vi "base info txt ransfer.vi"(11 "Base All Composition_edit":T1(array[cluster])) -> (3 "transposed array":string[][](array[string]))   [LabVIEW 2018]
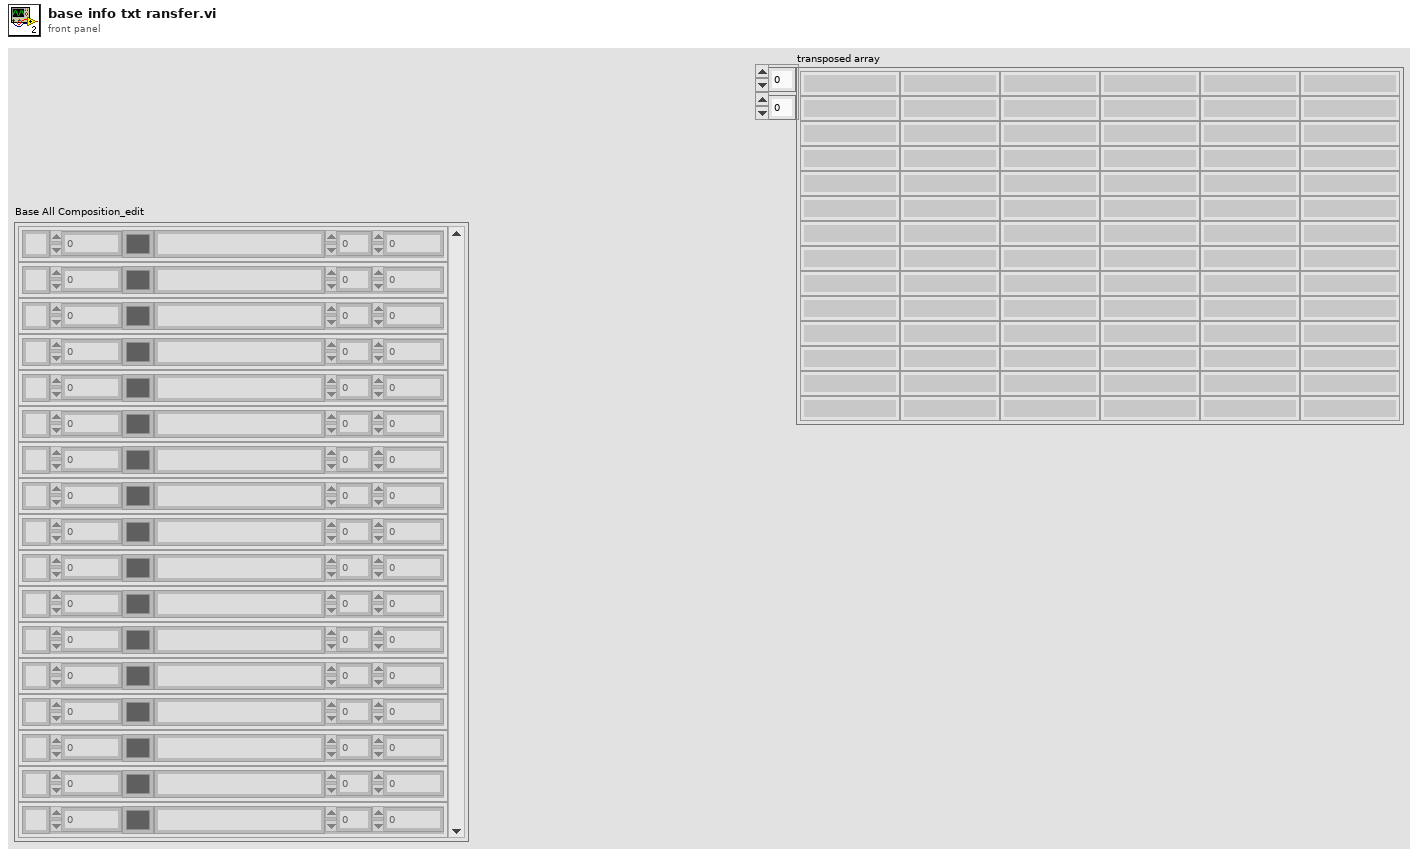
[diagram p1: front panel]
types:
  T1 = cluster{"Name":string, "Value":dbl, "Color":u32, "Name 2":string, "Value 2":dbl, "Value 3":dbl}[]
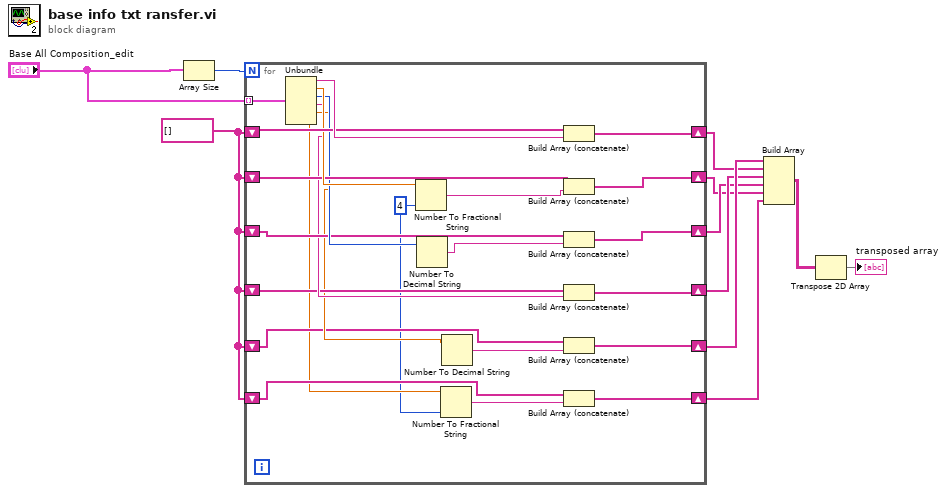
[diagram p0: block diagram]
diagram:
  w9 = string[] []
  n1 = Array Size(array="Base All Composition_edit") -> (size(s)=w11:i32)
  n2 = for {
    N: w11 -> [_]
    tunnel: "Base All Composition_edit" -> [w35] mode=indexing
    shift-right: [w34] -> w6
    shift-left: w9 -> [w32]
    shift-right: [w29] -> w3
    shift-left: w9 -> [w28]
    shift-right: [w25] -> w4
    shift-left: w9 -> [w24]
    shift-right: [w23] -> w5
    shift-left: w9 -> [w21]
    shift-right: [w20] -> w7
    shift-left: w9 -> [w16]
    shift-right: [w19] -> w8
    shift-left: w9 -> [w15]
    w13 = i16 4 ("precision (6)")
    n3 = Unbundle(w35) -> ("Name"=w33:string, "Value"=w31:dbl, "Color"=w27:u32, "Name 2"=w22:string, "Value 2"=w18:dbl, "Value 3"=w14:dbl)
    n4 = Number To Fractional String(number=w31, precision (6)=w13) -> (F-format string=w30:string)  [unwired: 2 in]
    n5 = Number To Decimal String(number=w27) -> (decimal integer string=w26:string)  [unwired: 1 in]
    n6 = Number To Fractional String(number=w14, precision (6)=w13) -> (F-format string=w12:string)  [unwired: 2 in]
    n7 = Number To Decimal String(number=w18) -> (decimal integer string=w17:string)  [unwired: 1 in]
    n8 = Build Array (concatenate)(w32, w33) -> (w34:string[])
    n9 = Build Array (concatenate)(w28, w30) -> (w29:string[])
    n10 = Build Array (concatenate)(w24, w26) -> (w25:string[])
    n11 = Build Array (concatenate)(w21, w22) -> (w23:string[])
    n12 = Build Array (concatenate)(w16, w17) -> (w20:string[])
    n13 = Build Array (concatenate)(w15, w12) -> (w19:string[])
  }
  n14 = Build Array(w7, w6, w5, w4, w3, w8) -> (w2:string[][])
  n15 = Transpose 2D Array(2D array=w2) -> (transposed array=→"transposed array":string[][])
